vi "Set PWM.Soft.vi"(8 "error in (no error)":errorcluster, 9 "Duty Cycle":dbl=0.5, 10 "PWM Freq":dbl=50.0, 11 "RPi PWM Pin in":T1=enum."GPIO12_PWM0_Pin32") -> (0 "error out":errorcluster, 1 "Actual Duty-Cycle":dbl, 2 "Actual Period":dbl=100.0, 3 "RPi PWM Pin out":T1=enum."GPIO12_PWM0_Pin32", 5 "PWM Timing":cluster{"PWM Range":u32, "PWM Data":u32})   [LabVIEW 2020, in "wiringPi.lvlib"]
doc: "<b>_______________________________________________________________</b>\n** Author: Juan José Villacorta\n** LabVIEW wrapper for C library <b> wiringPi </b>,\n** https://github.com/WiringPi/WiringPi\n<b>_______________________________________________________________</b>\n\nSet the PWM frequency and duty-cycle"
uses:
  wiringPi.lvlib
  <vilib>/ErrorRing/Error Ring.xnode
  <vilib>/Utility/error.llb/Error Cluster From Error Code.vi
  Type Defs/GPIO Pins.ctl
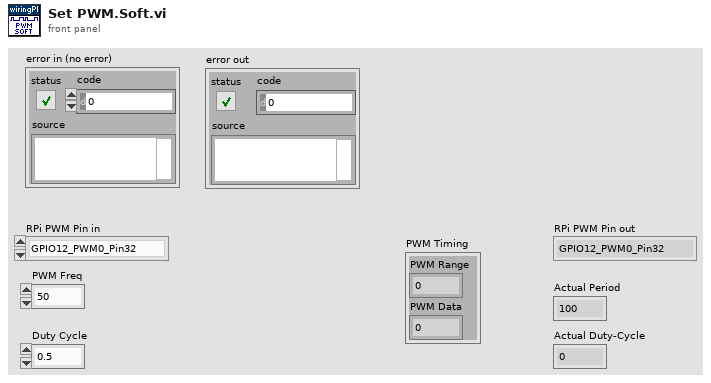
[diagram p1: front panel]
types:
  T1 = typedef "wiringPi.lvlib/GPIO Pins.ctl" = enum32{"GPIO0_I2C0_SDA_Pin27", "GPIO1_I2C0_SDA1_Pin28", "GPIO2_I2C1_SDA_Pin3", "GPIO3_I2C1_SCL_Pin5", "GPIO4_GPCLK0_Pin7", "GPIO5_GPCLK1_Pin29", "GPIO6_GPCLK2_Pin31", "GPIO7_SPI_CE1_N_Pin26", "GPIO8_SPI_CE0_N_Pin24", "GPIO9_SPI0_MISO_Pin21", "GPIO10_SPI0_MOSI_Pin19", "GPIO11_SPI0_CLK_Pin23", "GPIO12_PWM0_Pin32", "GPIO13_PWM1_Pin33", "GPIO14_TXD0_Pin8", "GPIO15_RXD0_Pin10", "GPIO16_Pin36", "GPIO17_Pin11", "GPIO18_PWM0_Pin12", "GPIO19_PWM1_Pin35", "GPIO20_GPCLK0_Pin38", "GPIO21_GPCLK1_Pin40", "GPIO22_Pin15", "GPIO23_Pin16", "GPIO24_Pin18", "GPIO25_Pin22", "GPIO26_Pin37", "GPIO27_Pin13"}
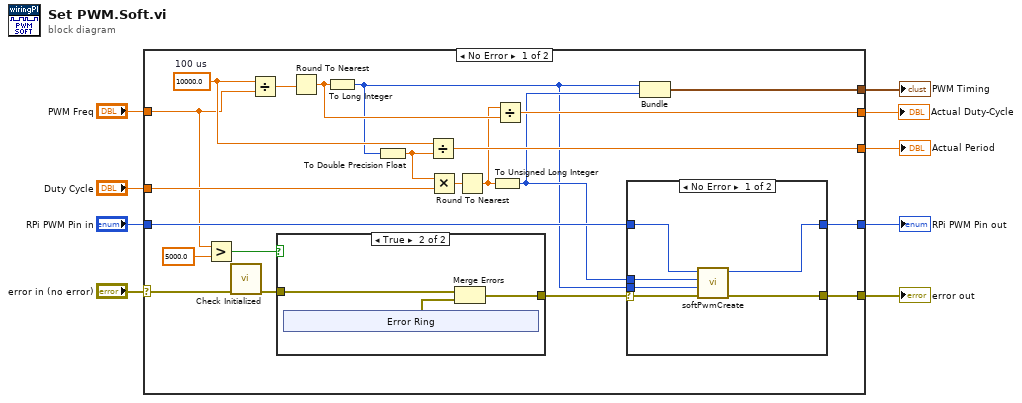
[diagram p0: block diagram]
diagram:
  n1 = case shown="No Error" "error in (no error)" {
    selector: "error in (no error)" -> [w11 w48]
    tunnel: [w30 w48] -> w9
    tunnel: "PWM Freq" -> [w14 _]
    tunnel: "RPi PWM Pin in" -> [w28 w49]
    tunnel: [w25 _] -> w6
    tunnel: [w20 _] -> w5
    tunnel: [w29 _] -> w4
    tunnel: [w27 w49] -> w2
    tunnel: "Duty Cycle" -> [w23 _]
    frame No Error {
      w22 = 10000.0  # 100 us
      n2 = Greater?(x=w14, y=5000.0) -> (0:w15:bool)
      n3 = call "Check Initialized.vi"("error in (no error)"=w11) -> ("error out"=w10:errorcluster)  [unwired: 10 in]
      n4 = Divide(x=w22, y=w14) -> (x/y=w26:dbl)
      n5 = case shown="True" w15 {
        tunnel: w10 -> [w31 w34]
        tunnel: [w31 w33] -> w16
        frame False {
        }
        frame True {
          n6 = xnode "Error Ring"() -> ("error out"=w32:errorcluster)
          n7 = Merge Errors(w34, w32) -> (w33:errorcluster)
        }
      }
      n8 = Round To Nearest(number=w26) -> (nearest integer value=w19:dbl)
      n9 = To Long Integer(number=w19) -> (32bit integer=w12:i32)
      n10 = To Double Precision Float(number=w12) -> (double precision float=w21:dbl)
      n11 = Divide(x=w22, y=w21) -> (x/y=w25:dbl)
      n12 = Multiply(x=w21, y=w23) -> (x*y=w24:dbl)
      n13 = Round To Nearest(number=w24) -> (nearest integer value=w18:dbl)
      n14 = To Unsigned Long Integer(number=w18) -> (unsigned 32bit integer=w17:u32)
      n15 = Divide(x=w18, y=w19) -> (x/y=w20:dbl)
      n16 = case shown="No Error" w16 {
        selector: w16 -> [w45 w47]
        tunnel: [w44 w47] -> w30
        tunnel: w28 -> [w43 w46]
        tunnel: [w40 w46] -> w27
        tunnel: w17 -> [w42 _]
        tunnel: w12 -> [w41 _]
        frame No Error {
          n17 = call "softPwmCreate.vi"("error in (no error)"=w45, "Range"=w41, "Value"=w42, "RPi Pin"=w43) -> ("error out"=w44:errorcluster, "RPi Pin out"=w40:T1)  [unwired: 6 in]
        }
        frame Error {
        }
      }
      n18 = Bundle(w12, w17) -> (w29:cluster{i32, u32})  [unwired: 1 in]
    }
    frame Error {
    }
  }
  "error out" <- w9
  "RPi PWM Pin out" <- w2
  "Actual Period" <- w6
  "Actual Duty-Cycle" <- w5
  "PWM Timing" <- w4
